vi "Func - get function name.vi"() -> (0 "found":bool, 1 "FuncVI name":string, 2 "Func name":string)   [LabVIEW 2021]
doc: "This VI returns a name of function and a name of FuncVI if it's in the FuncVI hierarchy.\n\nFor more information, see help for this VI.\n\n::: CalcExpress Toolkit :::\nCopyright (c) 2000-2026 Konstantin Shifershteyn. All rights reserved."
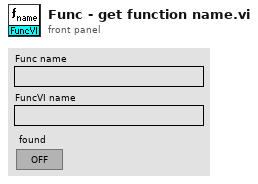
[diagram p1: front panel]
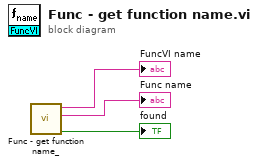
[diagram p0: block diagram]
diagram:
  n1 = call "Func - get function name_.vi"() -> ("found"=→"found":bool, "FuncVI name"=→"Func name":string, "Func name"=→"FuncVI name":string)  [unwired: 9 in]
